vi "VIH Project Tree - Shortcut Menu Handler.vi"(6 "Menu Tag":string, 8 "Coords":T1, 9 "MenuRef":refnum<k9>, 10 "Project Tree":T2, 11 "Event Type":T3) -> (3 "States spec":string)   [LabVIEW 2014]
doc: "::: VI Helpeks :::\nCopyright (c) 2000-2026 Konstantin Shifershteyn. All rights reserved."
uses:
  <vilib>/event_ctls.llb/lveventtype.ctl
  VIH Project Tree Typedef - Tree Refnum.ctl
  <vilib>/Utility/miscctls.llb/LVPoint32TypeDef.ctl
  VIH Project Tree Typedef - Tree Item Type.ctl
  _VIH Support Library.llb/VIH Utility - MENU - Create Menu (String).vi
panel:
  # "VI Helpeks\nCopyright (c) 2012-2026 Konstantin Shifershteyn"
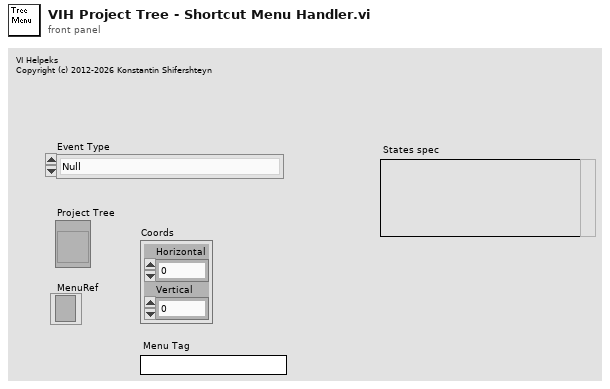
[diagram p1: front panel]
types:
  T1 = typedef "LVPoint32TypeDef.ctl" = cluster{"Horizontal":i32, "Vertical":i32}
  T2 = typedef "VIH Project Tree Typedef - Tree Refnum.ctl" = refnum<vi>
  T3 = typedef "lveventtype.ctl" = enum32{"Null", "Timeout", "Annotation Menu Selection", "Annotation Menu Selection?", "App Instance Close", "App Instance Close?", "Autoscale Range Change", "Bookmark Info Change", "Cell Edit", "Cell Edit?", "Cursor Grab", "Cursor Grab?", "Cursor Menu Selection", "Cursor Menu Selection?", "Cursor Move", "Cursor Release", "Data Change", "Direction Change", "Display State Change", "Drag Ended", "Drag Enter", "Drag Leave", "Drag Over", "Drag Source Update", "Drag Starting", "Drag Starting?", "Drop", "Exec State Change", "Key Down", "Key Down?", "Key Repeat", "Key Repeat?", "Key Up", "Listbox Double Click", "Menu Activation?", "Menu Selection (App)", "Menu Selection? (App)", "Menu Selection (User)", "Mouse Down", "Mouse Down?", "Mouse Enter", "Mouse Leave", "Mouse Move", "Mouse Up", "Mouse Wheel", "NI Security User Change (App)", "Pane Size", "Panel Close", "Panel Close?", "Panel Resize", "Plot Attribute Change", "Scale Range Change", "Shortcut Menu Activation?", "Shortcut Menu Selection (App)", "Shortcut Menu Selection? (App)", "Shortcut Menu Selection (User)", "Tree Double Click", "Tree Drag", "Tree Drag?", "Tree Drop", "Tree Drop?", "Tree Item Close", "Tree Item Close?", "Tree Item Open", "Tree Item Open?", "User Event", "Value Change"}
  T4 = typedef "VIH Project Tree Typedef - Tree Item Type.ctl" = enum32{"<Invalid>", "Project", "Proj Files", "Proj Rules", "File Group", "Rule Group", "Any File", "LV Func", ".mnu", ".mnu (dyn)", ".vi", ".vi (dyn)", ".vit", ".vit (dyn)", ".ctl", ".ctl (dyn)", ".ctt", ".ctt (dyn)", "polyVI", "polyVI (dyn)", "expVI", "expVI (dyn)", "HTML", "PolyVI Inst"}
  T5 = typedef "VIH - CHM Project - HHP Generation Params Cluster.ctl" = cluster{"HHP_Template":enum16{"default", "custom"}, "HHP_Template_CustomPath":path, "HHP_Target":enum16{"default", "custom"}, "HHP_Target_CustomPath":path, "HHP_CreateTOC":bool, "HHP_CreateIDX":bool, "HHP_DefaultTopic":enum16{"auto", "custom"}, "HHP_DefaultTopic_CustomPath":path, "CHM_Filename":path, "HHP_AutoBuild":bool, "CHM_AutoBuild":bool}
  T6 = typedef "VIH HelpGen Typedef - Cluster - File Rule.ctl" = cluster{"OutName":string, "BuildHelp":T7, "Source Paths":T8, "Target Paths":T9, "DscrMode":T10, "Description":string, "Control Rules":T11[], "Flags":T13, "Ctl_DscrMode":T10, "Ctl_ClustMembers":T7, "Ctl_EnumValues":T7, "MenuItemIcons":T7, "%Comments":string, "DetailsMode":T10, "DetailsText":string, "ProductInfoMode":T7, "ProductInfoText":string}
  T7 = typedef "VIH HelpGen Typedef - Enum - Default,Enable,Disable.ctl" = enum16{"Default", "Enable", "Disable"}
  T8 = typedef "VIH HelpGen Typedef - Cluster - File Rule - Source Paths.ctl" = cluster{"CSS Files":path[], "JS Files":path[], "Html Template":path}
  T9 = typedef "VIH HelpGen Typedef - Cluster - File Rule - Target Paths.ctl" = cluster{"HTML Dir":path, "Image Dir":path, "CSS Dir":path, "JS Dir":path}
  T10 = typedef "VIH HelpGen Typedef - Enum - Description Mode.ctl" = enum16{"Default", "Description", "Description1", "Description2", "Custom", "None"}
  T11 = typedef "VIH HelpGen Typedef - Cluster - Control Rule.ctl" = cluster{"CtrlID":string, "CustomRule":bool, "DscrMode":T10, "Description":string, "ClusterMembers":T7, "EnumValues":T7, "EnumValDscr":T12[], "CustomName":string}
  T12 = typedef "VIH HelpGen Typedef - Cluster - Enum Value Info.ctl" = cluster{"Value":ext, "String":string, "Description":string}
  T13 = typedef "VIH HelpGen Typedef - Cluster - Group Rule - Flags.ctl" = cluster{"Override CSS Files":bool, "Override JS Files":bool, "Override Ctl Rules":bool}
  T14 = typedef "VIH HelpGen Typedef - Palette - Item Type Enum.ctl" = enum32{"<Invalid>", "<unknown>", "VI", "Menu", "LV Func", "Express VI", "Poly VI", "CTL", "HTML"}
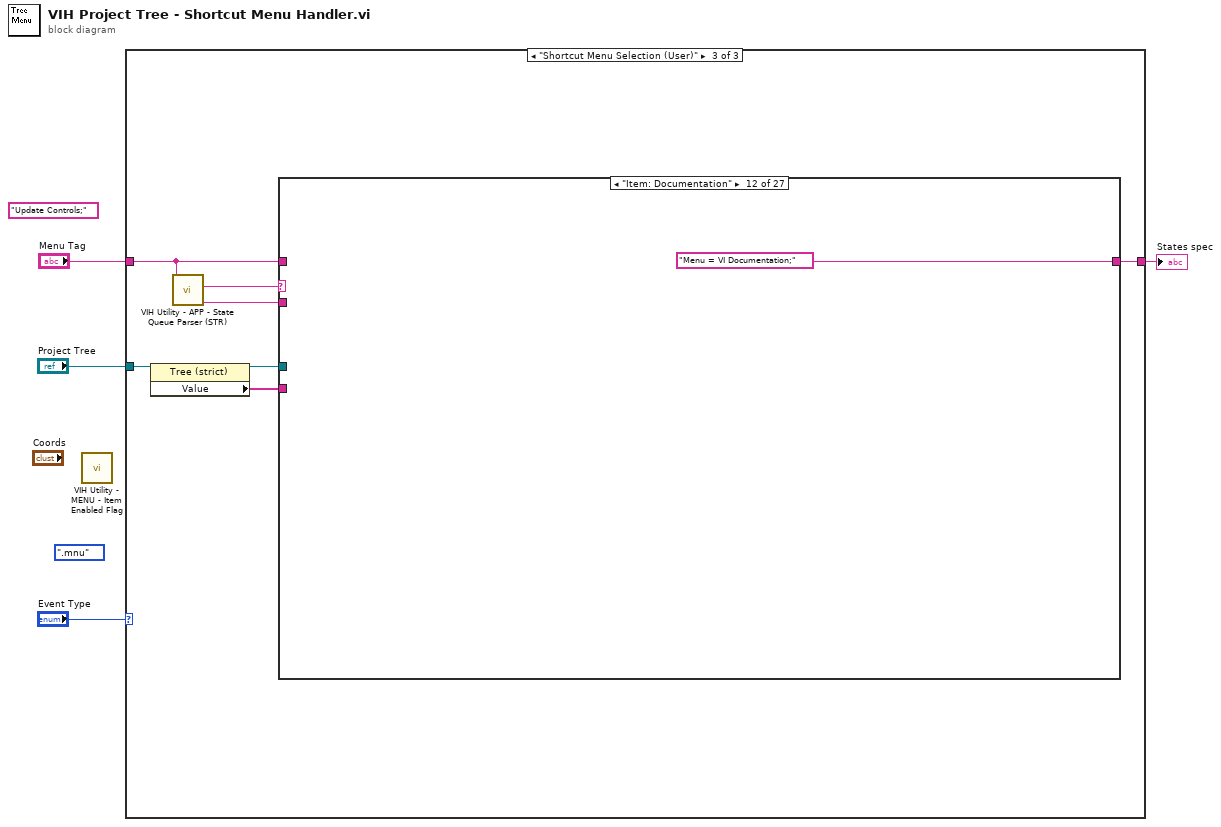
[diagram p0: block diagram]
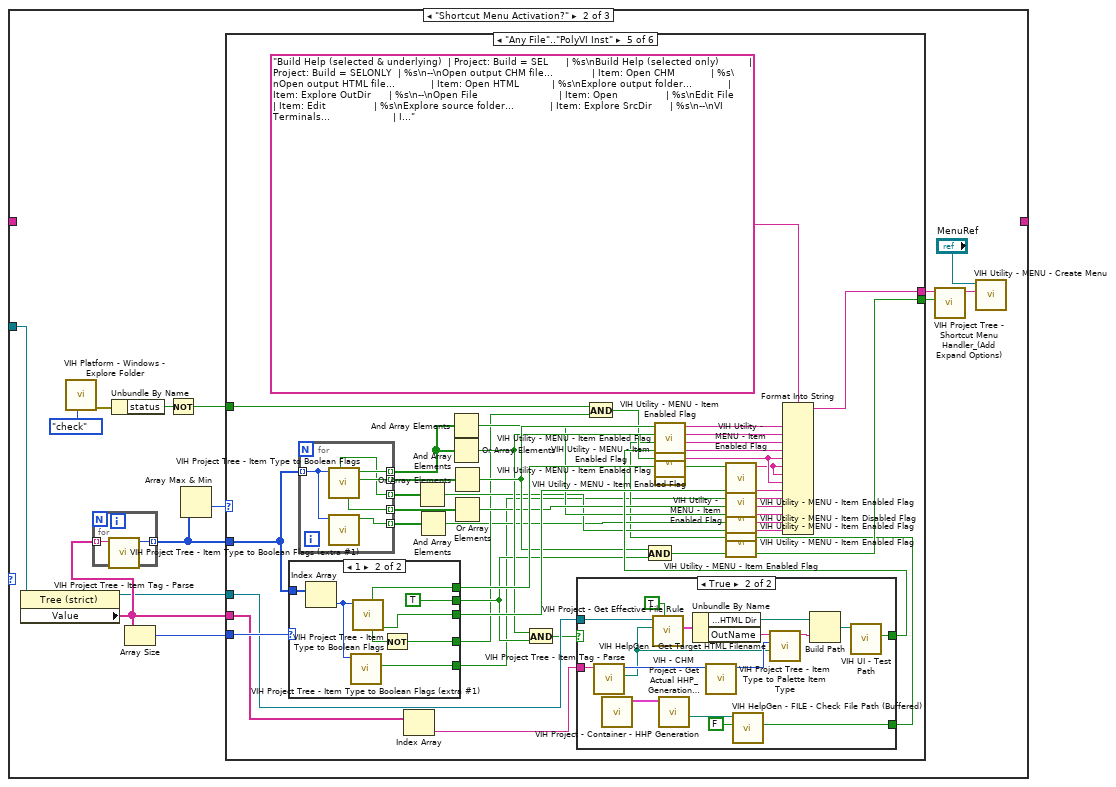
[diagram p3: hidden frame]
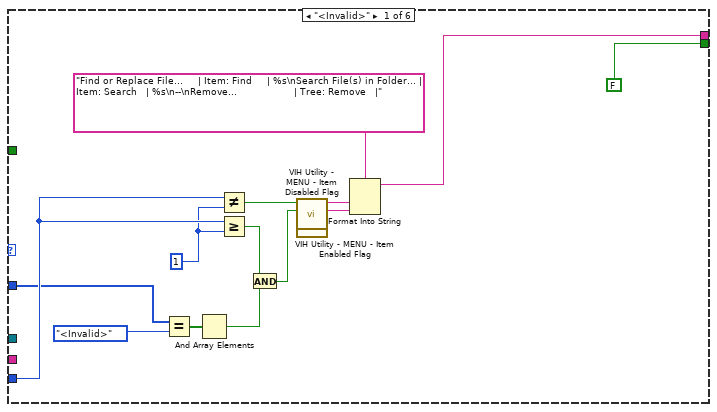
[diagram p4: hidden frame]
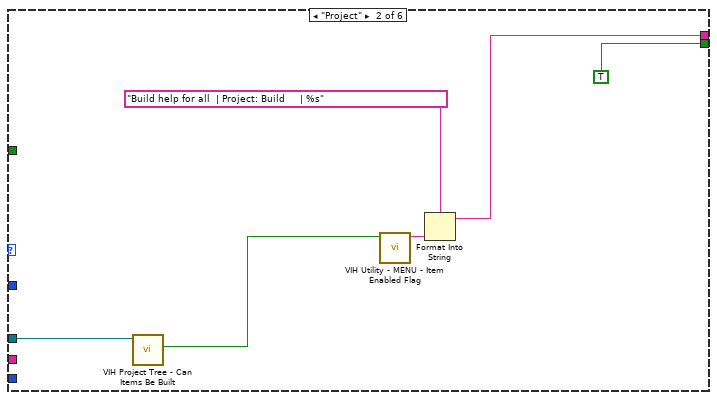
[diagram p5: hidden frame]
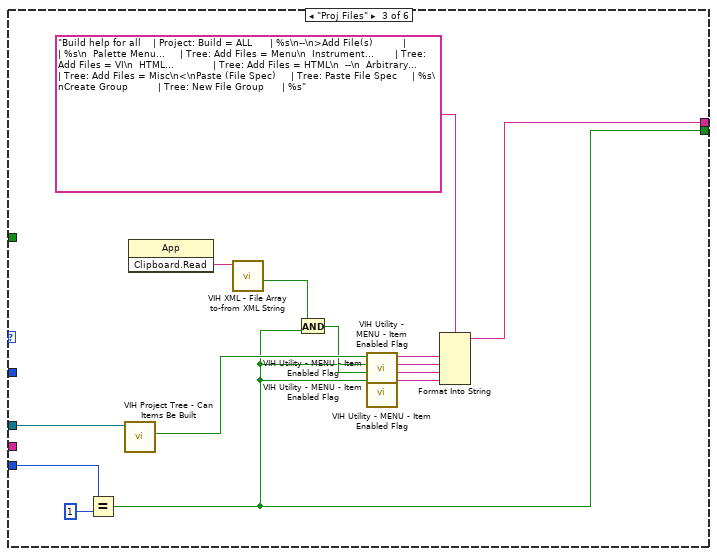
[diagram p6: hidden frame]
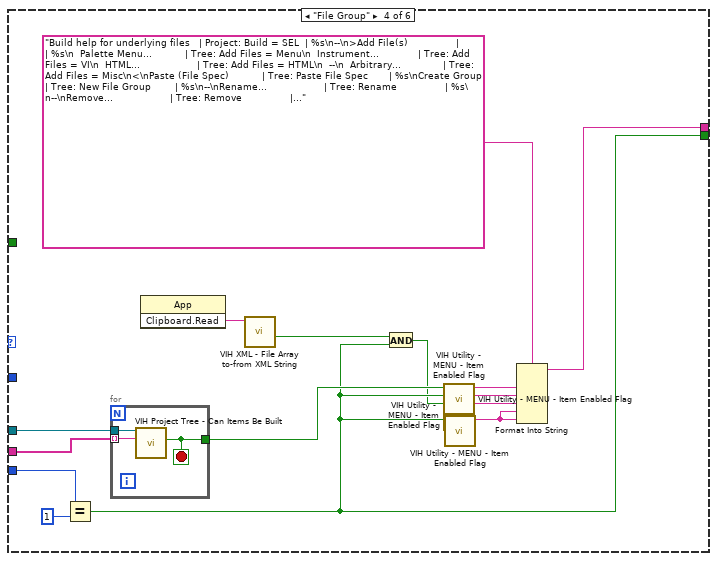
[diagram p7: hidden frame]
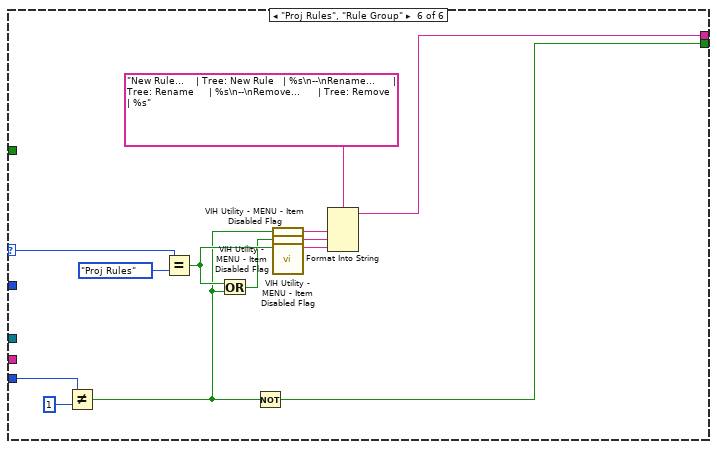
[diagram p10: hidden frame]
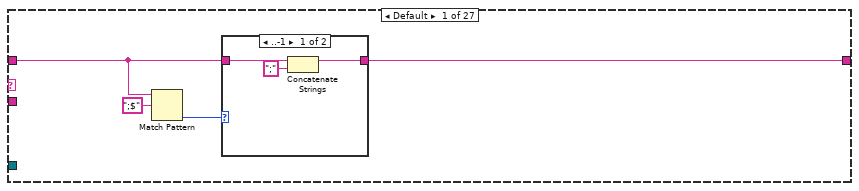
[diagram p11: hidden frame]
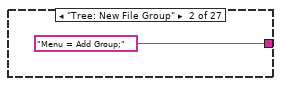
[diagram p13: hidden frame]
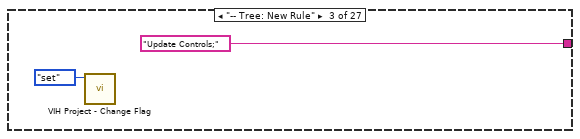
[diagram p14: hidden frame]
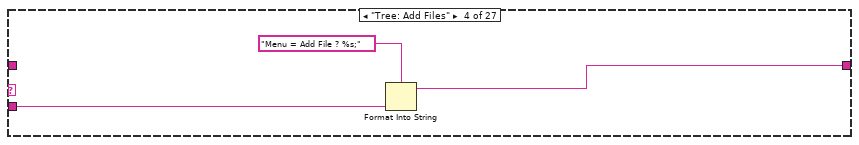
[diagram p15: hidden frame]
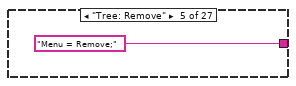
[diagram p16: hidden frame]
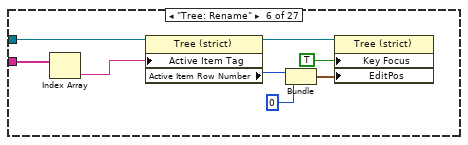
[diagram p17: hidden frame]
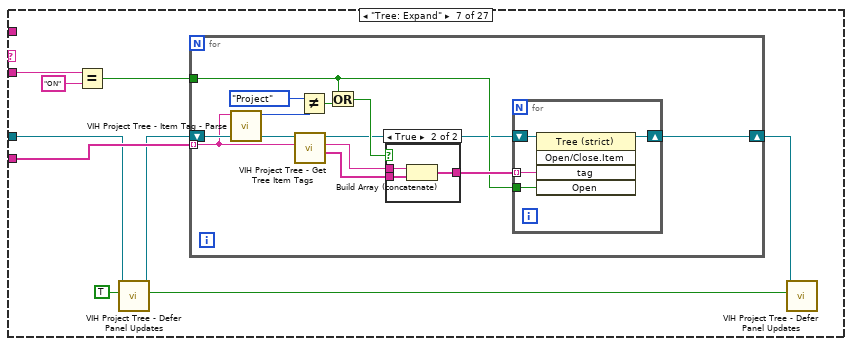
[diagram p18: hidden frame]
diagram:
  (unwired) "Update Controls;" ("Menu Tag")
  (unwired) VIH_Project_Tree_Typedef_-_Tree_Item_Type.".mnu" ("Item Type")
  n1 = call "VIH Utility - MENU - Item Enabled Flag.vi"() -> ()  [unwired: 11 in, 1 out]
  n2 = case shown="\"Shortcut Menu Selection (User)\"" "Event Type" {
    tunnel: "Project Tree" -> [_ w18 w160]
    tunnel: [_ _ w158] -> w2
    tunnel: "Menu Tag" -> [_ _ w162]
    frame Default {
    }
    frame "Shortcut Menu Activation?" {
      n3 = property class="Tree (strict)"(reference=w18) -> (reference out=w13:T2, "Value"=w14:string[])  [unwired: 1 in, 1 out]
      n4 = call "VIH Platform - Windows - Explore Folder.vi"("cmd (run)"=enum16{"run", "check"}."check") -> ("error out"=w7:errorcluster)  [unwired: 10 in]
      n5 = for {
        tunnel: w14 -> [w20] mode=indexing
        tunnel: [w19] -> w16 mode=indexing
        n6 = call "VIH Project Tree - Item Tag - Parse.vi"("Tree Item Tag"=w20) -> ("Item Type"=w19:T4)  [unwired: 8 in, 2 out]
      }
      n7 = Unbundle By Name(w7) -> ("status"=w6:bool)
      n8 = Array Size(array=w14) -> (size(s)=w15:i32)
      n9 = Not(x=w6) -> (.not. x?=w5:bool)
      n10 = Array Max & Min(array=w16) -> (min value=w17:T4)  [unwired: 3 out]
      n11 = case shown="\"Any File\"..\"PolyVI Inst\"" w17 {
        selector: w17 -> [_ _ _ _ _ w155]
        tunnel: w16 -> [w22 _ _ _ w99 _]
        tunnel: w15 -> [w31 _ w52 w67 w110 w150]
        tunnel: w14 -> [_ _ _ w65 w100 _]
        tunnel: w13 -> [_ w37 w48 w66 w101 _]
        tunnel: [w23 w39 w51 w62 w103 w146] -> w11
        tunnel: [FALSE TRUE w42 w57 w102 w144] -> w9
        tunnel: w5 -> [_ _ _ _ w85 _]
        frame "<Invalid>" {
          w30 = 1 ("y")
          n12 = Equal?(x=w22, y=VIH_Project_Tree_Typedef_-_Tree_Item_Type."<Invalid>" ("Item Type")) -> (x = y?=w27:bool[])
          n13 = And Array Elements(Boolean array=w27) -> (logical AND=w25:bool)
          n14 = Not Equal?(x=w31, y=w30) -> (x != y?=w32:bool)
          n15 = Greater Or Equal?(x=w31, y=w30) -> (x >= y?=w26:bool)
          n16 = And(x=w26, y=w25) -> (x .and. y?=w24:bool)
          n17 = call "VIH Utility - MENU - Item Disabled Flag.vi"("Disable?"=w32) -> ("Disable flag"=w33:string)  [unwired: 10 in]
          n18 = call "VIH Utility - MENU - Item Enabled Flag.vi"("Enable?"=w24) -> ("Disable flag"=w29:string)  [unwired: 10 in]
          n19 = Format Into String(format string="Find or Replace File...     | Item: Find     | %s\nSearch File(s) in Folder... | Item: Search   | %s\n--\nRemove...                   | Tree: Remove   |", w33, w29) -> (resulting string=w23:string)  [unwired: 2 in, 1 out]
        }
        frame "Project" {
          n20 = call "VIH Project Tree - Can Items Be Built.vi"("Project Tree"=w37) -> ("Can be built"=w36:bool)  [unwired: 7 in, 3 out]
          n21 = call "VIH Utility - MENU - Item Enabled Flag.vi"("Enable?"=w36) -> ("Disable flag"=w35:string)  [unwired: 10 in]
          n22 = Format Into String(format string="Build help for all  | Project: Build     | %s", w35) -> (resulting string=w39:string)  [unwired: 2 in, 1 out]
        }
        frame "Proj Files" {
          n23 = Equal?(x=w52, y=1) -> (x = y?=w42:bool)
          n24 = call "VIH Project Tree - Can Items Be Built.vi"("Project Tree"=w48) -> ("Can be built"=w49:bool)  [unwired: 7 in, 3 out]
          n25 = invoke class="App" method="Clipboard.Read"() -> ("Read Clipbrd"=w44:string)  [unwired: 3 in, 2 out]
          n26 = call "VIH XML - File Array to-from XML String.vi"("XML in"=w44) -> ("available"=w41:bool)  [unwired: 7 in, 3 out]
          n27 = And(x=w41, y=w42) -> (x .and. y?=w43:bool)
          n28 = call "VIH Utility - MENU - Item Enabled Flag.vi"("Enable?"=w49) -> ("Disable flag"=w50:string)  [unwired: 10 in]
          n29 = call "VIH Utility - MENU - Item Enabled Flag.vi"("Enable?"=w42) -> ("Disable flag"=w47:string)  [unwired: 10 in]
          n30 = call "VIH Utility - MENU - Item Enabled Flag.vi"("Enable?"=w43) -> ("Disable flag"=w46:string)  [unwired: 10 in]
          n31 = call "VIH Utility - MENU - Item Enabled Flag.vi"("Enable?"=w42) -> ("Disable flag"=w45:string)  [unwired: 10 in]
          n32 = Format Into String(format string="Build help for all    | Project: Build = ALL      | %s\n--\n>Add File(s)          |                           | %s\n  Palette Menu...     | Tree: Add Files = Menu\n  Instrument...       | Tree: Add Files = VI\n  HTML...             | Tree: Add Files = HTML\n  --\n  Arbitrary...        | Tree: Add Files = Misc\n<\nPaste (File Spec)     | Tree: Paste File Spec     | %s\nCreate Group          | Tree: New File Group      | %s", w50, w47, w46, w45) -> (resulting string=w51:string)  [unwired: 2 in, 1 out]
        }
        frame "File Group" {
          n33 = Equal?(x=w67, y=1) -> (x = y?=w57:bool)
          n34 = for {
            tunnel: w66 -> [w72]
            tunnel: w65 -> [w71] mode=indexing
            tunnel: [w70] -> w64
            stop <- w70 stop-if-true
            n35 = call "VIH Project Tree - Can Items Be Built.vi"("Parent Item Tag (Root)"=w71, "Project Tree"=w72) -> ("Can be built"=w70:bool)  [unwired: 6 in, 3 out]
          }
          n36 = invoke class="App" method="Clipboard.Read"() -> ("Read Clipbrd"=w61:string)  [unwired: 3 in, 2 out]
          n37 = call "VIH XML - File Array to-from XML String.vi"("XML in"=w61) -> ("available"=w56:bool)  [unwired: 7 in, 3 out]
          n38 = And(x=w56, y=w57) -> (x .and. y?=w55:bool)
          n39 = call "VIH Utility - MENU - Item Enabled Flag.vi"("Enable?"=w64) -> ("Disable flag"=w63:string)  [unwired: 10 in]
          n40 = call "VIH Utility - MENU - Item Enabled Flag.vi"("Enable?"=w57) -> ("Disable flag"=w60:string)  [unwired: 10 in]
          n41 = call "VIH Utility - MENU - Item Enabled Flag.vi"("Enable?"=w55) -> ("Disable flag"=w58:string)  [unwired: 10 in]
          n42 = call "VIH Utility - MENU - Item Enabled Flag.vi"("Enable?"=w57) -> ("Disable flag"=w59:string)  [unwired: 10 in]
          n43 = Format Into String(format string="Build help for underlying files   | Project: Build = SEL  | %s\n--\n>Add File(s)                |                             | %s\n  Palette Menu...           | Tree: Add Files = Menu\n  Instrument...             | Tree: Add Files = VI\n  HTML...                   | Tree: Add Files = HTML\n  --\n  Arbitrary...              | Tree: Add Files = Misc\n<\nPaste (File Spec)           | Tree: Paste File Spec       | %s\nCreate Group                | Tree: New File Group        | %s\n--\nRename...                   | Tree: Rename                | %s\n--\nRemove...                   | Tree: Remove                | ", w63, w60, w58, w59, w59) -> (resulting string=w62:string)  [unwired: 2 in, 1 out]
        }
        frame "Any File".."PolyVI Inst" {
          n44 = case shown="1" w110 {
            tunnel: w99 -> [_ w137]
            tunnel: [_ w135] -> w109
            tunnel: [_ w134] -> w108
            tunnel: [_ TRUE] -> w84
            tunnel: [_ w132] -> w81
            tunnel: [_ w130] -> w74
            frame Default {
            }
            frame 1 {
              n45 = Index Array(array=w137) -> (element=w131:T4)  [unwired: 1 in]
              n46 = call "VIH Project Tree - Item Type to Boolean Flags (extra #1).vi"("Item Type"=w131) -> ("Can be documented"=w130:bool)  [unwired: 9 in, 1 out]
              n47 = call "VIH Project Tree - Item Type to Boolean Flags.vi"("Item Type"=w131) -> ("VI with Conpane"=w134:bool, "Built In Function"=w133:bool, "Can be opened"=w135:bool)  [unwired: 4 in, 4 out]
              n48 = Not(x=w133) -> (.not. x?=w132:bool)
            }
          }
          n49 = for {
            tunnel: w99 -> [w139] mode=indexing
            tunnel: [w143] -> w91 mode=indexing
            tunnel: [w142] -> w98 mode=indexing
            tunnel: [w141] -> w94 mode=indexing
            tunnel: [w140] -> w86 mode=indexing
            tunnel: [w138] -> w79 mode=indexing
            n50 = call "VIH Project Tree - Item Type to Boolean Flags.vi"("Item Type"=w139) -> ("Palette menu"=w142:bool, "Can be built"=w143:bool, "Built In Function"=w141:bool, "Can be Removed"=w140:bool)  [unwired: 4 in, 3 out]
            n51 = call "VIH Project Tree - Item Type to Boolean Flags (extra #1).vi"("Item Type"=w139) -> ("Can have Qualified name"=w138:bool)  [unwired: 9 in, 1 out]
          }
          n52 = Index Array(array=w100) -> (element=w106:string)  [unwired: 1 in]
          n53 = And Array Elements(Boolean array=w86) -> (logical AND=w88:bool)
          n54 = And Array Elements(Boolean array=w79) -> (logical AND=w78:bool)
          n55 = And Array Elements(Boolean array=w91) -> (logical AND=w89:bool)
          n56 = Or Array Elements(Boolean array=w91) -> (logical OR=w95:bool)
          n57 = Or Array Elements(Boolean array=w98) -> (logical OR=w97:bool)
          n58 = Or Array Elements(Boolean array=w94) -> (logical OR=w93:bool)
          n59 = And(x=w95, y=w84) -> (x .and. y?=w96:bool)
          n60 = case shown="True" w96 {
            tunnel: [_ w121] -> w107
            tunnel: w101 -> [_ w120]
            tunnel: w106 -> [_ w119]
            tunnel: [_ w114] -> w76
            frame False {
            }
            frame True {
              n61 = call "VIH Project Tree - Item Tag - Parse.vi"("Tree Item Tag"=w119) -> ("Item File Path"=w118:path, "Item Type"=w128:T4)  [unwired: 8 in, 1 out]
              n62 = call "VIH Project - Container - HHP Generation.vi"() -> ("HHP_Generation out"=w117:T5)  [unwired: 11 in]
              n63 = call "VIH Project - Get Effective File Rule.vi"("Ignore Control Rules (F)"=TRUE, "File Path"=w118, "Project Tree"=w120) -> ("Effective File Rule"=w123:T6)  [unwired: 5 in, 3 out]
              n64 = call "VIH - CHM Project - Get Actual HHP_Generation Params.vi"("HHP_Generation"=w117) -> ("CHM File Absolute Path"=w115:path)  [unwired: 8 in, 2 out]
              n65 = Unbundle By Name(w123) -> ("Target Paths.HTML Dir"=w126:path, "OutName"=w125:string)
              n66 = call "VIH Project Tree - Item Type to Palette Item Type.vi"("Tree Item Type"=w128) -> ("Item/File Type"=w129:T14)  [unwired: 9 in, 1 out]
              n67 = call "VIH HelpGen - FILE - Check File Path (Buffered).vi"("Force Update (T)"=FALSE, "File Path"=w115) -> ("Good path"=w114:bool)  [unwired: 8 in, 1 out]
              n68 = call "VIH HelpGen - Get Target HTML Filename.vi"("Item File Path"=w118, "Item Type"=w129, "HTML Filename in"=w125) -> ("HTML Fileame out"=w127:string)  [unwired: 7 in, 1 out]
              n69 = Build Path(base path=w126, name or relative path=w127) -> (appended path=w122:path)
              n70 = call "VIH UI - Test Path.vi"("Path"=w122) -> ("Good Path"=w121:bool)  [unwired: 7 in, 3 out]
            }
          }
          n71 = And(x=w85, y=w81) -> (x .and. y?=w83:bool)
          n72 = And(x=w97, y=w84) -> (x .and. y?=w102:bool)
          n73 = call "VIH Utility - MENU - Item Enabled Flag.vi"("Enable?"=w97) -> ("Disable flag"=w112:string)  [unwired: 10 in]
          n74 = call "VIH Utility - MENU - Item Enabled Flag.vi"("Enable?"=w95) -> ("Disable flag"=w111:string)  [unwired: 10 in]
          n75 = call "VIH Utility - MENU - Item Enabled Flag.vi"("Enable?"=w76) -> ("Disable flag"=w75:string)  [unwired: 10 in]
          n76 = call "VIH Utility - MENU - Item Enabled Flag.vi"("Enable?"=w107) -> ("Disable flag"=w104:string)  [unwired: 10 in]
          n77 = call "VIH Utility - MENU - Item Enabled Flag.vi"("Enable?"=w83) -> ("Disable flag"=w82:string)  [unwired: 10 in]
          n78 = call "VIH Utility - MENU - Item Enabled Flag.vi"("Enable?"=w109) -> ("Disable flag"=w80:string)  [unwired: 10 in]
          n79 = call "VIH Utility - MENU - Item Enabled Flag.vi"("Enable?"=w108) -> ("Disable flag"=w105:string)  [unwired: 10 in]
          n80 = call "VIH Utility - MENU - Item Enabled Flag.vi"("Enable?"=w74) -> ("Disable flag"=w73:string)  [unwired: 10 in]
          n81 = call "VIH Utility - MENU - Item Disabled Flag.vi"("Disable?"=w93) -> ("Disable flag"=w92:string)  [unwired: 10 in]
          n82 = call "VIH Utility - MENU - Item Enabled Flag.vi"("Enable?"=w89) -> ("Disable flag"=w90:string)  [unwired: 10 in]
          n83 = call "VIH Utility - MENU - Item Enabled Flag.vi"("Enable?"=w78) -> ("Disable flag"=w77:string)  [unwired: 10 in]
          n84 = call "VIH Utility - MENU - Item Enabled Flag.vi"("Enable?"=w88) -> ("Disable flag"=w87:string)  [unwired: 10 in]
          n85 = Format Into String(format string="Build Help (selected & underlying)  | Project: Build = SEL      | %s\nBuild Help (selected only)          | Project: Build = SELONLY  | %s\n--\nOpen output CHM file...             | Item: Open CHM            | %s\nOpen output HTML file...            | Item: Open HTML           | %s\nExplore output folder...            | Item: Explore OutDir      | %s\n--\nOpen File                           | Item: Open                | %s\nEdit File                           | Item: Edit                | %s\nExplore source folder...            | Item: Explore SrcDir      | %s\n--\nVI Terminals...                     | Item: Terminals           | %s\nVI Documentation...                 | Item: Documentation       | %s\n--\n> Copy to Clipboard                 |                           | %s\n  File Spec                         | Item: Copy File Spec\n  Reference to the file             | Item: Copy Link           | %s\n  --\n  File path                         | Item: Copy Path\n  File name                         | Item: Copy Filename\n  Qualified VI name                 | Item: Copy Qualified Name | %s\n<\n--\nRemove...                           | Tree: Remove              | %s", w112, w111, w75, w104, w82, w80, w80, w82, w105, w73, w92, w90, w77, w87) -> (resulting string=w103:string)  [unwired: 2 in, 1 out]
        }
        frame "Proj Rules", "Rule Group" {
          n86 = Not Equal?(x=w150, y=1) -> (x != y?=w145:bool)
          n87 = Equal?(x=w155, y=VIH_Project_Tree_Typedef_-_Tree_Item_Type."Proj Rules") -> (x = y?=w153:bool)
          n88 = Or(x=w153, y=w145) -> (x .or. y?=w152:bool)
          n89 = Not(x=w145) -> (.not. x?=w144:bool)
          n90 = call "VIH Utility - MENU - Item Disabled Flag.vi"("Disable?"=w145) -> ("Disable flag"=w149:string)  [unwired: 10 in]
          n91 = call "VIH Utility - MENU - Item Disabled Flag.vi"("Disable?"=w152) -> ("Disable flag"=w147:string)  [unwired: 10 in]
          n92 = call "VIH Utility - MENU - Item Disabled Flag.vi"("Disable?"=w153) -> ("Disable flag"=w148:string)  [unwired: 10 in]
          n93 = Format Into String(format string="New Rule...    | Tree: New Rule   | %s\n--\nRename...      | Tree: Rename     | %s\n--\nRemove...      | Tree: Remove     | %s", w149, w147, w148) -> (resulting string=w146:string)  [unwired: 2 in, 1 out]
        }
      }
      n94 = call "VIH Project Tree - Shortcut Menu Handler_(Add Expand Options).vi"("Ena Expand/Collapse"=w9, "Menu dscr"=w11) -> ("Menu dscr out"=w10:string)  [unwired: 9 in]
      n95 = call-poly "VIH Utility - MENU - Create Menu.vi"("Menu Description"=w10, "menu"="MenuRef") -> ()  [unwired: 8 in, 2 out]
    }
    frame "Shortcut Menu Selection (User)" {
      n96 = property class="Tree (strict)"(reference=w160) -> (reference out=w159:T2, "Value"=w161:string[])  [unwired: 1 in, 1 out]
      n97 = call "VIH Utility - APP - State Queue Parser (STR).vi"("input queue"=w162) -> ("state parameters"=w157:string, "state"=w163:string)  [unwired: 5 in, 2 out]
      n98 = case shown="\"Item: Documentation\"" w163 {
        tunnel: [w164 "Menu = Add Group;" "Update Controls;" ("Menu Tag") w176 "Menu = Remove;" ("Menu Tag") _ _ _ "Menu = Open Source File;" "EXEC = Menu = Edit Source File;" "Menu = VI Terminals;" "Menu = VI Documentation;" "Menu = Open Output Help;" "Menu = Open CHM ? SEL;" w222 w234 _ _ _ _ _ _ "Menu = Copy File Spec;" "Menu = Paste File Spec;" _ _ _] -> w158
        tunnel: w162 -> [w165 _ _ _ _ _ _ _ _ _ _ _ _ _ _ _ _ _ _ _ _ _ _ _ _ _ _]
        tunnel: w159 -> [_ _ _ _ _ w186 w192 _ _ _ _ _ _ _ w227 w238 _ _ _ _ _ _ _ _ _ _ w289]
        tunnel: w161 -> [_ _ _ _ _ w180 w195 _ _ _ _ _ _ _ w228 w237 _ w249 w256 w264 w277 _ _ _ _ w284 w293]
        tunnel: w157 -> [_ _ _ w177 _ _ w194 _ _ _ _ _ _ _ _ _ _ _ _ _ _ _ _ _ _ _ _]
        frame Default {
          n99 = Match Pattern(string=w165, regular expression=";$") -> (offset past match=w166:i32)  [unwired: 1 in, 3 out]
          n100 = case shown="..-1" w166 {
            tunnel: w165 -> [w170 w171]
            tunnel: [w169 w171] -> w164
            frame ..-1 {
              n101 = Concatenate Strings(w170, ";" ("string")) -> (w169:string)
            }
            frame 0.. {
            }
          }
        }
        frame "Tree: New File Group" {
        }
        frame "-- Tree: New Rule" {
          n102 = call "VIH Project - Change Flag.vi"("cmd (get)"=enum16{"get", "set", "reset"}."set") -> ()  [unwired: 9 in, 2 out]
        }
        frame "Tree: Add Files" {
          n103 = Format Into String(format string="Menu = Add File ? %s;", w177) -> (resulting string=w176:string)  [unwired: 2 in, 1 out]
        }
        frame "Tree: Remove" {
        }
        frame "Tree: Rename" {
          n104 = Index Array(array=w180) -> (element=w179:string)  [unwired: 1 in]
          n105 = property class="Tree (strict)"(reference=w186, "Active Item Tag"=w179) -> (reference out=w185:T2, "Active Item Row Number"=w183:i32)  [unwired: 1 in, 1 out]
          n106 = Bundle("Active Item Row Number"=w183, 0) -> (w182:cluster{"Active Item Row Number":i32, i32})  [unwired: 1 in]
          n107 = property class="Tree (strict)"(reference=w185, "Key Focus"=TRUE, "EditPos"=w182) -> ()  [unwired: 1 in, 2 out]
        }
        frame "Tree: Expand" {
          n108 = Equal?(x=w194, y="ON") -> (x = y?=w187:bool)
          n109 = call "VIH Project Tree - Defer Panel Updates.vi"("Defer Panel Updates (F)"=TRUE, "Project Tree"=w192) -> ("Previous Defer status"=w189:bool, "dup Project Tree"=w191:T2)  [unwired: 7 in, 1 out]
          n110 = for {
            tunnel: w195 -> [w204] mode=indexing
            shift-right: [w205] -> w190
            shift-left: w191 -> [w207]
            tunnel: w187 -> [w197]
            n111 = call "VIH Project Tree - Item Tag - Parse.vi"("Tree Item Tag"=w204) -> ("Item Type"=w203:T4)  [unwired: 8 in, 2 out]
            n112 = call "VIH Project Tree - Get Tree Item Tags.vi"("Parent Item Tag"=w204, "Project Tree"=w207) -> ("Child Item Tags"=w199:string[], "dup Parent Item Tag"=w200:string, "dup Project Tree"=w196:T2)  [unwired: 6 in, 1 out]
            n113 = Not Equal?(x=VIH_Project_Tree_Typedef_-_Tree_Item_Type."Project", y=w203) -> (x != y?=w201:bool)
            n114 = Or(x=w197, y=w201) -> (x .or. y?=w198:bool)
            n115 = case shown="True" w198 {
              tunnel: [w208 w211] -> w206
              tunnel: w200 -> [_ w210]
              tunnel: w199 -> [w208 w209]
              frame False {
              }
              frame True {
                n116 = Build Array (concatenate)(w210, w209) -> (w211:string[])
              }
            }
            n117 = for {
              tunnel: w206 -> [w214] mode=indexing
              tunnel: w197 -> [w213]
              shift-right: [w212] -> w205
              shift-left: w196 -> [w215]
              n118 = invoke class="Tree (strict)" method="Open/Close.Item"(reference=w215, "tag"=w214, "Open"=w213) -> (reference out=w212:T2)  [unwired: 2 in, 4 out]
            }
          }
          n119 = call "VIH Project Tree - Defer Panel Updates.vi"("Defer Panel Updates (F)"=w189, "Project Tree"=w190) -> ()  [unwired: 7 in, 3 out]
        }
        frame "----------------------------- 1" {
        }
        frame "Item: Open" {
        }
        frame "Item: Edit" {
          (unwired) "Menu = Edit Source File;"
        }
        frame "Item: Terminals" {
        }
        frame "Item: Documentation" {
        }
        frame "Item: Open HTML" {
        }
        frame "Item: Open CHM" {
        }
        frame "Item: Find" {
          n120 = Index Array(array=w228) -> (element=w226:string)  [unwired: 1 in]
          n121 = call "VIH Dialog - Find File on Disk.vi"("Tree Item Tag"=w226, "Project Tree"=w227) -> ("New Tree Item Tag"=w223:string, "dup Project Tree"=w225:T2)  [unwired: 6 in, 2 out]
          n122 = Empty String/Path?(string/path=w223) -> (empty?=w224:bool)
          n123 = case shown="False" w224 {
            tunnel: w225 -> [w232 _]
            tunnel: w223 -> [w230 _]
            tunnel: ["Update Controls;\nUpdate Toolbar: Warning;" ("Menu Tag") _] -> w222
            frame False {
              n124 = Build Array(w230) -> (w231:string[])
              n125 = property class="Tree (strict)"(reference=w232, "Value"=w231) -> (reference out=w233:T2)  [unwired: 1 in, 1 out]
              n126 = invoke class="Tree (strict)" method="Open/Close.Ensure Visible"(reference=w233, "tag"=w230) -> ()  [unwired: 2 in, 4 out]
            }
            frame True {
            }
          }
        }
        frame "Item: Search" {
          n127 = call "VIH Dialog - Search Files in Folder.vi"("Tree Item Tags"=w237, "Project Tree"=w238) -> ("Tree Item Tags out"=w235:string[], "dup Project Tree"=w236:T2)  [unwired: 6 in, 2 out]
          n128 = Empty Array?(array=w235) -> (empty?=w239:bool)
          n129 = case shown="False" w239 {
            tunnel: w236 -> [w242 _]
            tunnel: w235 -> [w241 _]
            tunnel: ["Update Controls;\nUpdate Toolbar: Warning;" ("Menu Tag") _] -> w234
            frame False {
              n130 = property class="Tree (strict)"(reference=w242, "Value"=w241) -> (reference out=w243:T2)  [unwired: 1 in, 1 out]
              n131 = disable-structure shown="Disabled" {
                disable-tunnel: w243 -> [w244 _]
                frame Disabled {
                  n132 = invoke class="Tree (strict)" method="Open/Close.Ensure Visible"(reference=w244) -> ()  [unwired: 3 in, 4 out]
                }
                frame Enabled {
                }
              }
            }
            frame True {
            }
          }
        }
        frame "----------------------------- 2" {
        }
        frame "Item: Copy Link" {
          n133 = for {
            tunnel: [w250] -> w247 mode=indexing
            tunnel: w249 -> [w251] mode=indexing
            n134 = call "VIH HelpGen - HREF - Build.vi"("Tree Item Tag"=w251) -> ("A HREF"=w250:string)  [unwired: 10 in]
          }
          n135 = call "VIH Utility - STR - Remove Empty Strings from 1D Array.vi"("String array in"=w247) -> ("String array out"=w246:string[])  [unwired: 9 in, 1 out]
          n136 = call "VIH Utility - STR - Remove Duplicated Strings from 1D Array.vi"("Array in"=w246) -> ("Array out"=w245:string[])  [unwired: 9 in, 1 out]
          n137 = call "VIH Utility - STR - String from 1D Str Array.vi"("Array in"=w245) -> ("String out"=w248:string)  [unwired: 6 in]
          n138 = invoke class="App" method="Clipboard.Write"("Param 0"=w248) -> ()  [unwired: 3 in, 4 out]
        }
        frame "Item: Copy Filename" {
          n139 = for {
            tunnel: [w257] -> w253 mode=indexing
            tunnel: w256 -> [w259] mode=indexing
            n140 = call "VIH Project Tree - Item Tag - Parse.vi"("Tree Item Tag"=w259) -> ("Item File Path"=w258:path)  [unwired: 8 in, 2 out]
            n141 = Strip Path(path=w258) -> (name=w257:string)  [unwired: 1 out]
          }
          n142 = call "VIH Utility - STR - Remove Empty Strings from 1D Array.vi"("String array in"=w253) -> ("String array out"=w254:string[])  [unwired: 9 in, 1 out]
          n143 = call "VIH Utility - STR - Remove Duplicated Strings from 1D Array.vi"("Array in"=w254) -> ("Array out"=w252:string[])  [unwired: 9 in, 1 out]
          n144 = call "VIH Utility - STR - String from 1D Str Array.vi"("Array in"=w252) -> ("String out"=w255:string)  [unwired: 6 in]
          n145 = invoke class="App" method="Clipboard.Write"("Param 0"=w255) -> ()  [unwired: 3 in, 4 out]
        }
        frame "Item: Copy Qualified Name" {
          n146 = for {
            tunnel: [w265] -> w261 mode=indexing
            tunnel: w264 -> [w267] mode=indexing
            n147 = call "VIH Project Tree - Item Tag - Parse.vi"("Tree Item Tag"=w267) -> ("Item File Path"=w266:path)  [unwired: 8 in, 2 out]
            n148 = call "VIH HelpGen - FILE - Get Qualified Filename.vi"("File Path"=w266) -> ("Qualified name"=w265:string)  [unwired: 9 in, 1 out]
          }
          n149 = call "VIH Utility - STR - Remove Empty Strings from 1D Array.vi"("String array in"=w261) -> ("String array out"=w262:string[])  [unwired: 9 in, 1 out]
          n150 = call "VIH Utility - STR - Remove Duplicated Strings from 1D Array.vi"("Array in"=w262) -> ("Array out"=w260:string[])  [unwired: 9 in, 1 out]
          n151 = call "VIH Utility - STR - String from 1D Str Array.vi"("Array in"=w260) -> ("String out"=w263:string)  [unwired: 6 in]
          n152 = invoke class="App" method="Clipboard.Write"("Param 0"=w263) -> ()  [unwired: 3 in, 4 out]
        }
        frame "Item: Copy Path" {
          n153 = for {
            tunnel: w277 -> [w279] mode=indexing
            tunnel: [w278] -> w270 mode=indexing
            n154 = call "VIH Project Tree - Item Tag - Parse.vi"("Tree Item Tag"=w279) -> ("Item File Path"=w278:path)  [unwired: 8 in, 2 out]
          }
          n155 = Build Array(path "", path "") -> (w275:path[])
          n156 = call "VIH Utility - FILE - Filter 1D Array of Paths.vi"("Action (keep instances)"=enum16{"keep instances", "remove instances"}."remove instances", "Instances"=w275, "Paths in"=w270) -> ("Paths out"=w272:path[])  [unwired: 4 in]
          n157 = call "VIH Utility - FILE - Remove Duplicated Paths from 1D Array.vi"("Array in"=w272) -> ("Array out"=w269:path[])  [unwired: 9 in, 1 out]
          n158 = Path To String(path=w269) -> (string=w268:string[])
          n159 = call "VIH Utility - STR - String from 1D Str Array.vi"("Array in"=w268) -> ("String out"=w276:string)  [unwired: 6 in]
          n160 = invoke class="App" method="Clipboard.Write"("Param 0"=w276) -> ()  [unwired: 3 in, 4 out]
        }
        frame "----------------------------- 3" {
        }
        frame "Item: Copy File Spec" {
        }
        frame "Tree: Paste File Spec" {
        }
        frame "----------------------------- 4" {
        }
        frame "Item: Explore SrcDir" {
          n161 = Index Array(array=w284) -> (element=w283:string)  [unwired: 1 in]
          n162 = call "VIH Project Tree - Item Tag - Parse.vi"("Tree Item Tag"=w283) -> ("Item File Path"=w282:path)  [unwired: 8 in, 2 out]
          n163 = call "VIH Platform - Windows - Explore Folder.vi"("cmd (run)"=enum16{"run", "check"}."run", "exe/doc/dir path"=w282) -> ("error out"=w286:errorcluster)  [unwired: 9 in]
          n164 = call <vilib>:"Simple Error Handler.vi"("error in (no error)"=w286) -> ()  [unwired: 4 in, 5 out]
        }
        frame "Item: Explore OutDir" {
          n165 = Index Array(array=w293) -> (element=w288:string)  [unwired: 1 in]
          n166 = call "VIH Project Tree - Item Tag - Parse.vi"("Tree Item Tag"=w288) -> ("Item File Path"=w290:path)  [unwired: 8 in, 2 out]
          n167 = call "VIH Project - Get Effective File Rule.vi"("Ignore Control Rules (F)"=TRUE, "File Path"=w290, "Project Tree"=w289) -> ("Effective File Rule"=w291:T6)  [unwired: 5 in, 3 out]
          n168 = Unbundle By Name(w291) -> ("Target Paths.HTML Dir"=w287:path)
          n169 = call "VIH Platform - Windows - Explore Folder.vi"("cmd (run)"=enum16{"run", "check"}."run", "exe/doc/dir path"=w287) -> ("error out"=w295:errorcluster)  [unwired: 9 in]
          n170 = call <vilib>:"Simple Error Handler.vi"("error in (no error)"=w295) -> ()  [unwired: 4 in, 5 out]
        }
      }
    }
  }
  "States spec" <- w2
